vi "SetClientComplexityv2.vi"() -> ()   [LabVIEW 2017]
uses:
  <vilib>/httpClient/POSTBuffer.vi
  <vilib>/httpClient/LabVIEWHTTPClient.lvlib
panel:
  out "body":string
  out "error out":errorcluster
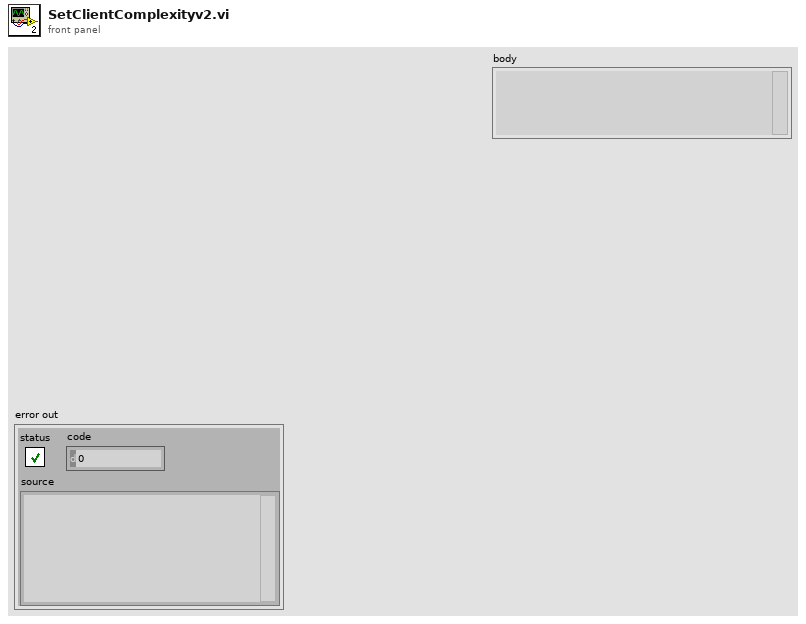
[diagram p1: front panel]
types:
  T1 = cluster{"req_action":string, "selector":string, "req_lang":string, "device":string, "type_descriptor":i16[]}
  T2 = cluster{"dbl_field":dbl, "string_field":string, "long_field":i64, "int_array_field":i32[]}
  T3 = typedef "LabVIEWHTTPClient.lvlib/ClientHandle.ctl" = refnum<k1>
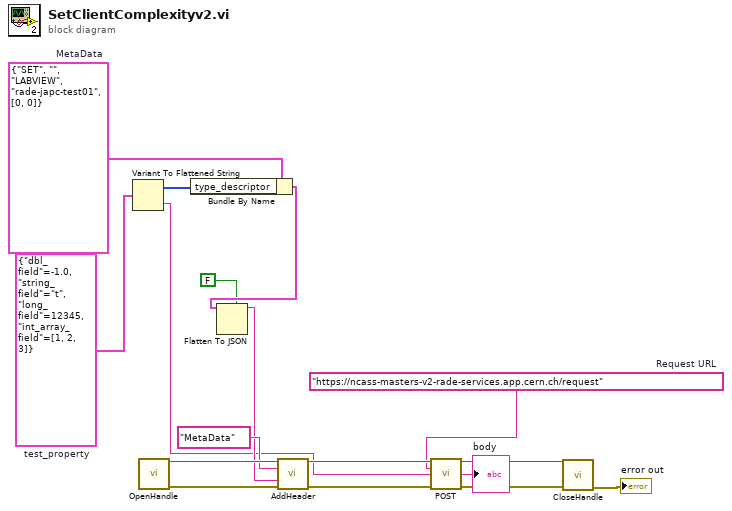
[diagram p0: block diagram]
diagram:
  w4 = "https://ncass-masters-v2-rade-services.app.cern.ch/request"  # Request URL
  w13 = T1 {"req_action"="SET", "selector"="", "req_lang"="LABVIEW", "device"="rade-japc-test01", "type_descriptor"=[0, 0]}  # MetaData
  w2 = T2 {"dbl_field"=-1.0, "string_field"="t", "long_field"=12345, "int_array_field"=[1, 2, 3]}  # test_property
  n1 = Variant To Flattened String(Variant=w2) -> (data string=w1:string, 1:w9:i16[])
  n2 = call <vilib>:"OpenHandle.vi"() -> ("client handle out"=w16:T3, "error out"=w17:errorcluster)  [unwired: 14 in]
  n3 = Bundle By Name(cluster=w13, "type_descriptor"=w9) -> (w12:T1)
  n4 = Flatten To JSON(enable LabVIEW extensions? (T)=FALSE, anything=w12) -> (JSON string=w10:string)  [unwired: 1 in, 1 out]
  n5 = call <vilib>:"AddHeader.vi"("client handle"=w16, "header"="MetaData", "value"=w10, "error in (no error)"=w17) -> ("client handle out"=w8:T3, "error out"=w7:errorcluster)  [unwired: 10 in]
  n6 = call-poly <vilib>:"POST.vi"("client handle"=w8, "url"=w4, "buffer"=w1, "error in (no error)"=w7) -> ("client handle out"=w6:T3, "body"=→"body":string, "error out"=w5:errorcluster)  [unwired: 8 in, 1 out]
  n7 = call <vilib>:"CloseHandle.vi"("client handle"=w6, "error in (no error)"=w5) -> ("error out"=→"error out":errorcluster)  [unwired: 13 in]
